vi "Check Protection.vi"(8 "error in (no error)":errorcluster, 10 "String in":string, 11 "SMC Protection in":refnum<class "SMC Protection.lvclass">) -> (0 "error out":errorcluster, 1 "Protection Error":errorcluster, 2 "String out":string, 3 "SMC Protection out":refnum<class "SMC Protection.lvclass">)   [LabVIEW 2026, in "Protections.lvlib" / "SMC Protection.lvclass"]
uses:
  SMC Protection.lvclass
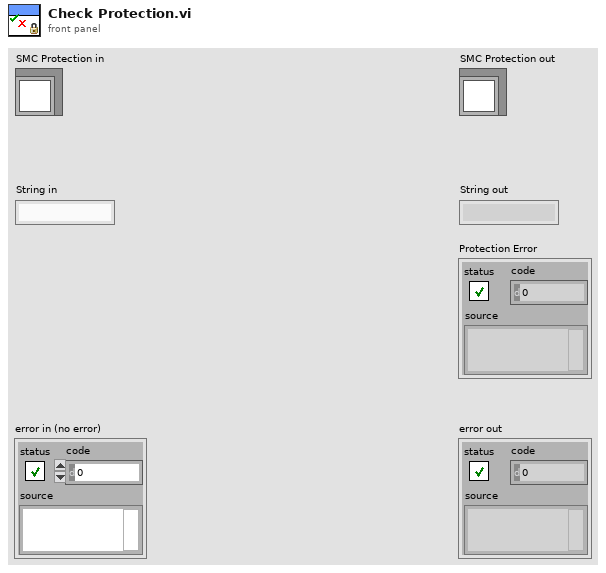
[diagram p1: front panel]
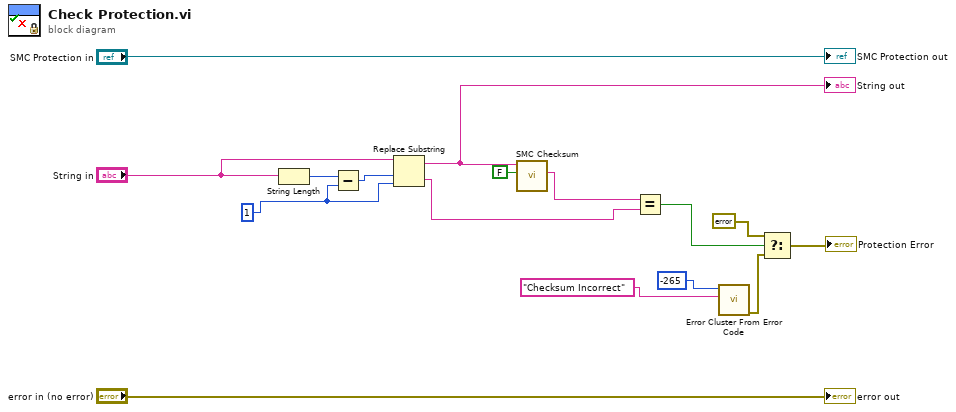
[diagram p0: block diagram]
diagram:
  w14 = 1
  n1 = String Length(string="String in") -> (length=w16:i32)
  n2 = Subtract(x=w16, y=w14) -> (x-y=w15:i32)
  n3 = Replace Substring(2:w14, 3:w15, 5:"String in") -> (0:w4:string, 1:w10:string)  [unwired: 1 in]
  "String out" <- w10
  n4 = call "SMC Checksum.vi"("Pad"=FALSE, "String in"=w10) -> ("Checksum String"=w3:string)  [unwired: 8 in, 1 out]
  n5 = Equal?(x=w3, y=w4) -> (x = y?=w5:bool)
  n6 = call <vilib>:"Error Cluster From Error Code.vi"("error message (\"\")"="Checksum Incorrect" ("error message (\"\")"), "error code (0)"=-265) -> ("error out"=w7:errorcluster)  [unwired: 7 in]
  n7 = Select(t=errorcluster {"status"=FALSE, "code"=0, "source"=""}, s=w5, f=w7) -> (s? t:f=→"Protection Error":errorcluster)
  "error out" <- "error in (no error)"
  "SMC Protection out" <- "SMC Protection in"
